vi "VM - Context Info.vi"(8 "error in":errorcluster, 11 "VC Handle":T2=-1) -> (0 "error out":errorcluster, 1 "Creator":string, 2 "VC Name":string, 3 "dup VC Handle":T2=-1, 5 "context life time":T1)   [LabVIEW 2021]
doc: "This VI returns information about the specified variable context. Refer to the VI help for more details.\n\n<b>VC Handle</b> control specifies the handle of a variable context.\n\n<b>VC Name</b> indicator returns the name of the variable context</b>.\n\n<b>Creator</b> indicator returns the name of the context creator.\n\n<b>Context life time</b> indicator returns the value specified as a context lifetime when the context was opened.\n\n::: CalcExpress Toolkit :::\nCopyright (c) 2000-2026 Konstantin Shifershteyn. All rights reserved."
uses:
  cetypes.llb/VarMan Variable Context Handle.ctl
  cetypes.llb/VarMan Context Life Time.ctl
  cetypes.llb/VarMan Error Code.ctl
  cersrc/celveng32.dll
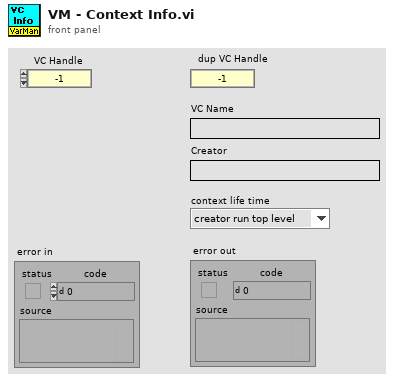
[diagram p1: front panel]
types:
  T1 = typedef "VarMan Context Life Time.ctl" = enum32{"creator run top level", "creator running ", "creator in memory", "untill closed"}
  T2 = typedef "VarMan Variable Context Handle.ctl" = i32
  T3 = typedef "VarMan Error Code.ctl" = u16
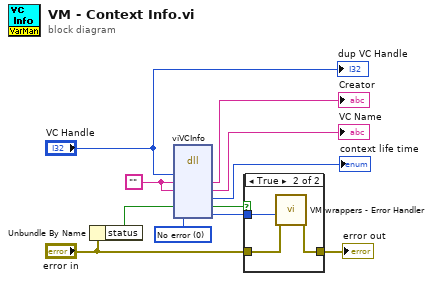
[diagram p0: block diagram]
diagram:
  w4 = T3 0 items=["No error", "Invalid variable type", "Variable not found", "Variable already exists", "Invalid context handle", "Input error", "Invalid data format", "No history attached", "History already attached", "Invalid history parameters", "Wrong variable name", "Wrong alias name", "Non-unique alias", "Alias not found", "No alias associated", "Alias already associated", "Wrong context name", "Non-unique context name", "Context name not found", "Invalid parameter", "Generic error", "Memory Full", "Unrecognized LV error", "Unknown error code"] ("VarMan error")
  w9 = "" ("Empty String Constant")
  n1 = Unbundle By Name("error in") -> ("status"=w6:bool)
  n2 = dll-call lib="C:/LV Projects/CalcExpress 40 LV2021/vi.lib/addons/CalcExpress/cersrc/celveng*.dll" fn="viVCInfo"("vch"="VC Handle", "Creator"=w9, "vcName"=w9, "errf"=w6, "errc"=w4) -> ("Creator"=→"Creator":string, "vcName"=→"VC Name":string, "context life time"=→"context life time":T1, "errf"=w5:bool, "errc"=w3:T3)  [unwired: 6 in, 2 out]
  n3 = case shown="True" w5 {
    tunnel: [w12 w15] -> w11
    tunnel: "error in" -> [w12 w14]
    tunnel: w3 -> [_ w13]
    frame False {
    }
    frame True {
      n4 = call "VM wrappers - Error Handler.vi"("error before"=w14, "VarMan error"=w13) -> ("error out"=w15:errorcluster)  [unwired: 8 in, 1 out]
    }
  }
  "error out" <- w11
  "dup VC Handle" <- "VC Handle"
